vi "RP1210 Read Detailed Version.vi"(8 "error in (no error)":errorcluster, 11 "nClientID":i16) -> (0 "error out":errorcluster, 1 "fpchFWVersionInfo":string, 2 "fpchDLLVersionInfo":string, 3 "fpchAPIVersionInfo":string, 5 "function return":i16)   [LabVIEW 2020, in "cansub_rp1210.lvlib"]
doc: "short __stdcall RP1210_ReadDetailedVersion(short nClientID, char *fpchAPIVersionInfo,\n char *fpchDLLVersionInfo, char *fpchFWVersionInfo);"
uses:
  cansub_rp1210.lvlib
  cansub_lv64.dll
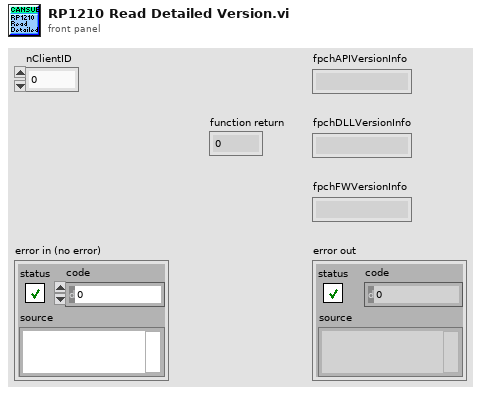
[diagram p1: front panel]
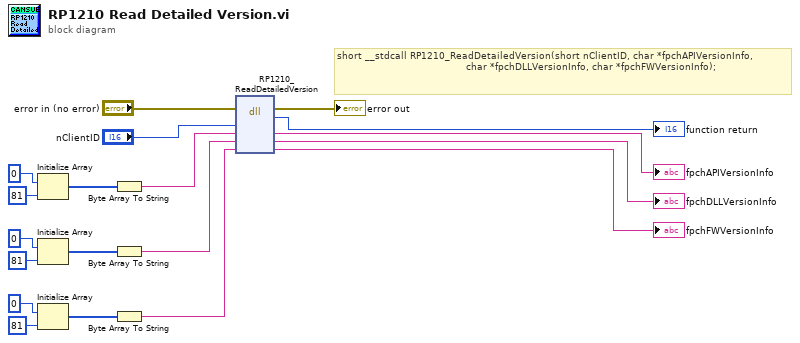
[diagram p0: block diagram]
diagram:
  # "short __stdcall RP1210_ReadDetailedVersion(short nClientID, char *fpchAPIVersionInfo,\n                                           char *fpchDLLVersionInfo, char *fpchFWVersionInfo);"
  n1 = Initialize Array(u8 0 ("element"), 81 ("dimension size")) -> (w17:u8[])
  n2 = Initialize Array(u8 0 ("element"), 81 ("dimension size")) -> (w12:u8[])
  n3 = Initialize Array(u8 0 ("element"), 81 ("dimension size")) -> (w7:u8[])
  n4 = Byte Array To String(unsigned byte array=w17) -> (string=w16:string)
  n5 = Byte Array To String(unsigned byte array=w12) -> (string=w11:string)
  n6 = Byte Array To String(unsigned byte array=w7) -> (string=w6:string)
  n7 = dll-call lib="C:/cansub-lv/library/cansub_lv*.*" fn="RP1210_ReadDetailedVersion"(error in="error in (no error)", "nClientID"="nClientID", "fpchAPIVersionInfo"=w16, "fpchDLLVersionInfo"=w11, "fpchFWVersionInfo"=w6) -> (error out=→"error out":errorcluster, "return type"=→"function return":i16, "fpchAPIVersionInfo"=→"fpchAPIVersionInfo":string, "fpchDLLVersionInfo"=→"fpchDLLVersionInfo":string, "fpchFWVersionInfo"=→"fpchFWVersionInfo":string)  [unwired: 3 in, 1 out]
